vi "Linear Fit (multiple).vi"(8 "error in (no error)":errorcluster, 9 "Type":enum16{"y vs x", "x vs y"}(ring), 11 "XY-data":cluster{"X-array":dbl[], "Y-array":dbl[]}[](array[cluster]) {"Y-array" format="%.2p"; "X-array" format="%.2p"}) -> (0 "error out":errorcluster, 2 "Best Fits":cluster{"X-array":dbl[], "Y-array":dbl[]}[](array[cluster]), 3 "XY-data out":cluster{"X-array":dbl[], "Y-array":dbl[]}[](array[cluster]) {"Y-array" format="%.2p"; "X-array" format="%.2p"}, 4 "slopes":dbl[](array[numeric]), 5 "Lower Bounds":cluster{"X-array":dbl[], "Y-array":dbl[]}[](array[cluster]), 6 "intercepts":dbl[](array[numeric]), 7 "Upper Bounds":cluster{"X-array":dbl[], "Y-array":dbl[]}[](array[cluster]))   [LabVIEW 2019, in "xy_utilities.lvlib"]
doc: "Performs a linear fit using linear LS algorithm.\n\nWire data to the data input to determine the polymorphic instance to use or manually select the instance."
uses:
  xy_utilities.lvlib
  Swap X and Y.vi
  Swap X and Y (single).vi
  <vilib>/Analysis/6fits.llb/Linear Fit Intervals.vi
  <vilib>/Analysis/6fits.llb/Confidence Interval (Linear).vi
  <vilib>/Analysis/6fits.llb/Linear Fit.vi
  <vilib>/Utility/error.llb/Error Cluster From Error Code.vi
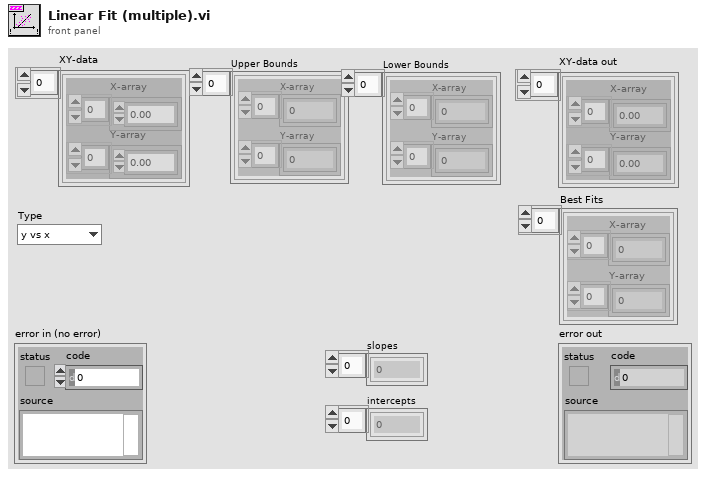
[diagram p1: front panel]
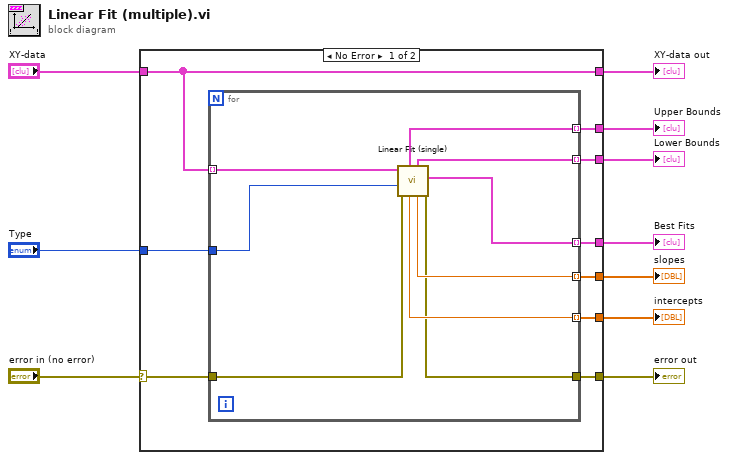
[diagram p0: block diagram]
diagram:
  n1 = case shown="No Error" "error in (no error)" {
    selector: "error in (no error)" -> [w11 w30]
    tunnel: [w19 w30] -> w9
    tunnel: "XY-data" -> [w12 w29]
    tunnel: [w12 w29] -> w7
    tunnel: "Type" -> [w18 _]
    tunnel: [w17 _] -> w5
    tunnel: [w16 _] -> w4
    tunnel: [w15 _] -> w3
    tunnel: [w14 _] -> w1
    tunnel: [w13 _] -> w2
    frame No Error {
      n2 = for {
        tunnel: w12 -> [w28] mode=indexing
        tunnel: w18 -> [w22]
        tunnel: [w27] -> w17 mode=indexing
        tunnel: [w25] -> w16 mode=indexing
        tunnel: [w26] -> w15 mode=indexing
        tunnel: [w24] -> w14 mode=indexing
        tunnel: [w23] -> w13 mode=indexing
        tunnel: [w21] -> w19
        tunnel: w11 -> [w20]
        n3 = call "Linear Fit (single).vi"("error in (no error)"=w20, "Type"=w22, "XY-data"=w28) -> ("error out"=w21:errorcluster, "Best Fit"=w27:cluster{"X-array":dbl[], "Y-array":dbl[]}, "slope"=w25:dbl, "Lower Bound"=w24:cluster{"X-array":dbl[], "Y-array":dbl[]}, "intercept"=w26:dbl, "Upper Bound"=w23:cluster{"X-array":dbl[], "Y-array":dbl[]})  [unwired: 2 in, 1 out]
      }
    }
    frame Error {
    }
  }
  "error out" <- w9
  "XY-data out" <- w7
  "Best Fits" <- w5
  "slopes" <- w4
  "intercepts" <- w3
  "Upper Bounds" <- w2
  "Lower Bounds" <- w1
